vi "Load SA Manual Setting.vi"(8 "error in (no error)":errorcluster caption="에러 입력(에러 없음)", 10 "SA Manual Param":T1={"Start Frequency"=0.0, "Stop Frequency"=0.0, "RBW"=0.0, "VBW"=0.0, "Sweep Point"=0, "Sweep Time"=0.0, "Atten Level"=0.0, "Detector Type"=enum."RMS", "Limit"=0.0}, 11 "Instrument Manager 입력":refnum<class "Instrument Manager.lvclass">) -> (0 "error out":errorcluster caption="에러 출력", 3 "Instrument Manager 출력":refnum<class "Instrument Manager.lvclass">)   [LabVIEW 2023, in "Instrument Manager.lvclass"]
uses:
  Instrument Manager.lvclass
  Type Definition/SA Manual Param.ctl
  Module/Spectrum Analyzer/TYPE DEFINITION/TYPE Detect Mode Select.ctl
  Instrument Manager.lvclass/Instrument Manager.ctl
  Module/Spectrum Analyzer/Spectrum Analyzer.lvlib
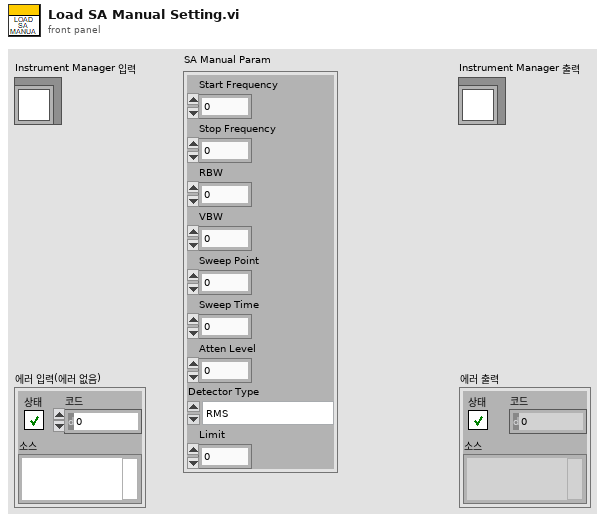
[diagram p1: front panel]
types:
  T1 = typedef "SA Manual Param.ctl" = cluster{"Start Frequency":dbl, "Stop Frequency":dbl, "RBW":dbl, "VBW":dbl, "Sweep Point":u32, "Sweep Time":dbl, "Atten Level":dbl, "Detector Type":T2, "Limit":dbl}
  T2 = typedef "Spectrum Analyzer.lvlib/TYPE Detect Mode Select.ctl" = enum16{"Det Auto (Normal)", "Auto Peak", "Positive Peak", "Negative Peak", "Sample", "RMS", "Average", "Quasipeak", "CISPR Average", "RMS Average"}
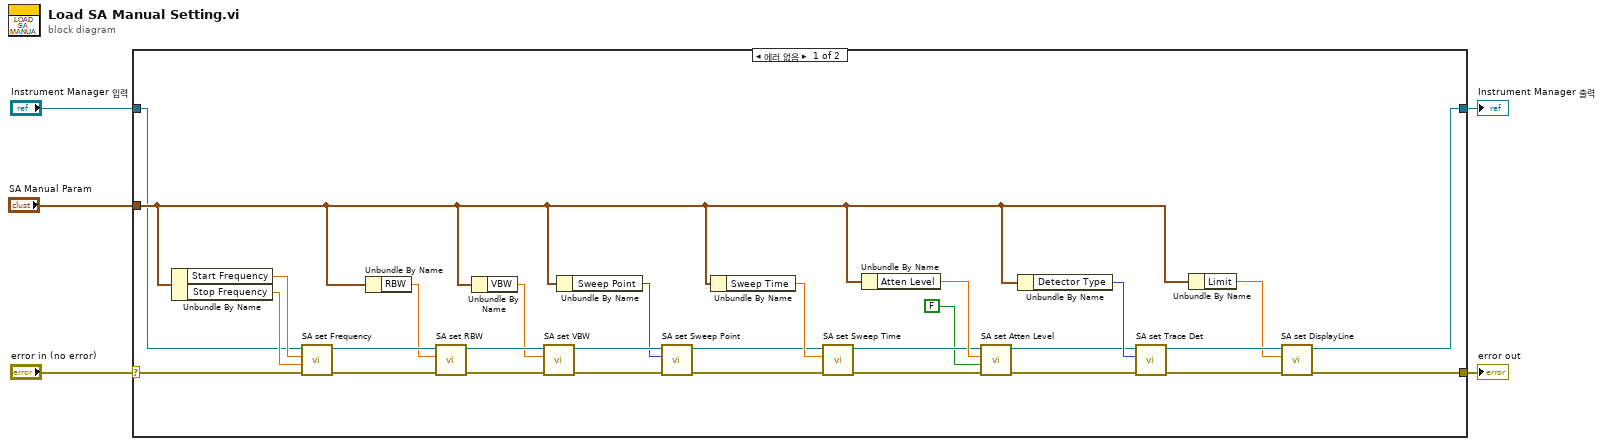
[diagram p0: block diagram]
diagram:
  n1 = case shown="에러 없음" "error in (no error)" {
    selector: "error in (no error)" -> [w23 w36]
    tunnel: [w10 w36] -> w4
    tunnel: [w6 w35] -> w2
    tunnel: "Instrument Manager 입력" -> [w7 w35]
    tunnel: "SA Manual Param" -> [w12 _]
    frame No Error {
      n2 = Unbundle By Name(w12) -> ("Start Frequency"=w27:dbl, "Stop Frequency"=w28:dbl)
      n3 = call "SA set Frequency.vi"("error in (no error)"=w23, "Stop"=w28, "Start"=w27, "Instrument Manager 입력"=w7) -> ("error out"=w34:errorcluster, "Instrument Manager 출력"=w31:refnum<class "Instrument Manager.lvclass">)  [unwired: 6 in]
      n4 = Unbundle By Name(w12) -> ("RBW"=w26:dbl)
      n5 = call "SA set RBW.vi"("error in (no error)"=w34, "BW Value (Hz)"=w26, "Instrument Manager 입력"=w31) -> ("error out"=w33:errorcluster, "Instrument Manager 출력"=w30:refnum<class "Instrument Manager.lvclass">)  [unwired: 7 in]
      n6 = Unbundle By Name(w12) -> ("VBW"=w25:dbl)
      n7 = call "SA set VBW.vi"("error in (no error)"=w33, "BW Value (Hz)"=w25, "Instrument Manager 입력"=w30) -> ("error out"=w32:errorcluster, "Instrument Manager 출력"=w29:refnum<class "Instrument Manager.lvclass">)  [unwired: 7 in]
      n8 = Unbundle By Name(w12) -> ("Sweep Point"=w24:u32)
      n9 = call "SA set Sweep Point.vi"("error in (no error)"=w32, "Sweep Point"=w24, "Instrument Manager 입력"=w29) -> ("error out"=w21:errorcluster, "Instrument Manager 출력"=w18:refnum<class "Instrument Manager.lvclass">)  [unwired: 7 in]
      n10 = Unbundle By Name(w12) -> ("Sweep Time"=w22:dbl)
      n11 = call "SA set Sweep Time.vi"("error in (no error)"=w21, "Sweep Time(sec)"=w22, "Instrument Manager 입력"=w18) -> ("error out"=w19:errorcluster, "Instrument Manager 출력"=w17:refnum<class "Instrument Manager.lvclass">)  [unwired: 7 in]
      n12 = Unbundle By Name(w12) -> ("Atten Level"=w20:dbl)
      n13 = call "SA set Atten Level.vi"("error in (no error)"=w19, "Auto?"=FALSE, "Attenuation"=w20, "Instrument Manager 입력"=w17) -> ("error out"=w14:errorcluster, "Instrument Manager 출력"=w13:refnum<class "Instrument Manager.lvclass">)  [unwired: 6 in]
      n14 = Unbundle By Name(w12) -> ("Detector Type"=w15:T2)
      n15 = call "SA set Trace Det.vi"("error in (no error)"=w14, "Detector Type"=w15, "Instrument Manager 입력"=w13) -> ("error out"=w11:errorcluster, "Instrument Manager 출력"=w9:refnum<class "Instrument Manager.lvclass">)  [unwired: 7 in]
      n16 = Unbundle By Name(w12) -> ("Limit"=w8:dbl)
      n17 = call "SA set DisplayLine.vi"("error in (no error)"=w11, "Amplitude"=w8, "Instrument Manager 입력"=w9) -> ("error out"=w10:errorcluster, "Instrument Manager 출력"=w6:refnum<class "Instrument Manager.lvclass">)  [unwired: 7 in]
    }
    frame Error {
    }
  }
  "error out" <- w4
  "Instrument Manager 출력" <- w2
